vi "Calc phase increase and offset.vi"(6 "Phase offset (deg)":dbl, 7 "# of DDS":i32=4, 8 "error in (no error)":errorcluster, 9 "resolution (32bit)":i32=32, 10 "fclk (MHz)":dbl=800000000.0 format="%#_6p", 11 "f_generated (MHz)":dbl=10.0) -> (0 "error out":errorcluster, 2 "Phase out":fxp<+,64,64>[](array[numeric]), 3 "delta":i64)   [LabVIEW 2025]
doc: "Calculates Phase Increment (\"pinc\") information for DDS core."
panel:
  out "Numeric":dbl
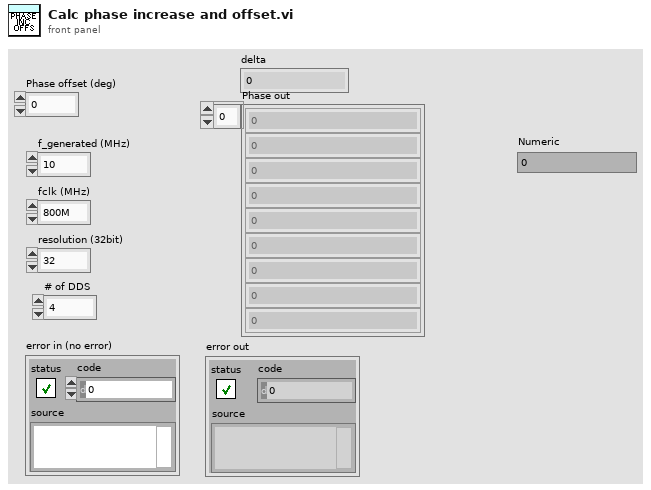
[diagram p1: front panel]
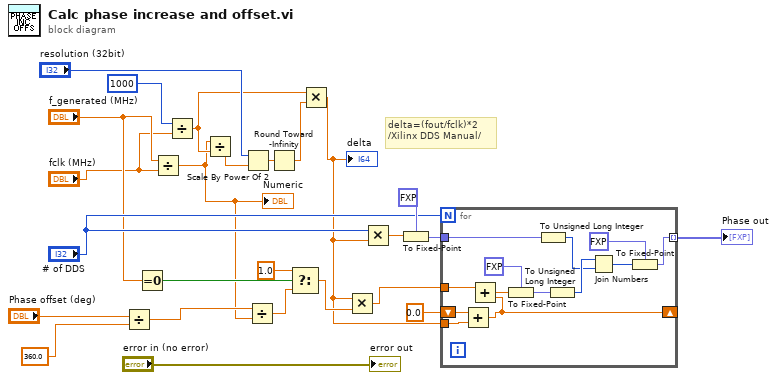
[diagram p0: block diagram]
diagram:
  # "delta=(fout/fclk)*2\n/Xilinx DDS Manual/"
  n1 = Divide(x="Phase offset (deg)", y=360.0) -> (x/y=w17:dbl)
  n2 = Equal To 0?(x="f_generated (MHz)") -> (x = 0?=w11:bool)
  n3 = Divide(x="f_generated (MHz)", y="fclk (MHz)") -> (x/y=w2:dbl)
  "Numeric" <- w2
  n4 = Divide(x=1000, y="fclk (MHz)") -> (x/y=w3:dbl)
  n5 = Divide(x=w2, y=w3) -> (x/y=w7:dbl)
  n6 = Scale By Power Of 2(n="resolution (32bit)", x=w7) -> (x*2^n=w21:dbl)
  n7 = Divide(x=w17, y=w2) -> (x/y=w12:dbl)
  n8 = Round Toward -Infinity(1:w21) -> (0:w4:dbl)
  n9 = Select(t=1.0, s=w11, f=w12) -> (s? t:f=w10:dbl)
  n10 = Multiply(x=w3, y=w4) -> (x*y=w6:dbl)
  "delta" <- w6
  n11 = Multiply(x=w6, y=w10) -> (x*y=w16:dbl)
  n12 = Multiply(x="# of DDS", y=w6) -> (x*y=w14:dbl)
  n13 = To Fixed-Point(fixed-point type=fxp<+,32,32> 0.0 ("pinc_in0"), number=w14) -> (fixed-point=w22:fxp<+,32,32>)
  n14 = for {
    N: "# of DDS" -> [_]
    tunnel: w22 -> [w33]
    tunnel: [w27] -> w19 mode=indexing
    tunnel: w6 -> [w38]
    shift-right: [w35] -> _
    shift-left: 0.0 -> [w36]
    tunnel: w16 -> [w34]
    n15 = Add(x=w36, y=w38) -> (x+y=w35:dbl)
    n16 = Add(x=w34, y=w35) -> (x+y=w26:dbl)
    n17 = To Fixed-Point(fixed-point type=fxp<+,32,32> 0.0 ("pinc_in0"), number=w26) -> (fixed-point=w32:fxp<+,32,32>)
    n18 = To Unsigned Long Integer(number=w33) -> (unsigned 32bit integer=w30:u32)
    n19 = To Unsigned Long Integer(number=w32) -> (unsigned 32bit integer=w31:u32)
    n20 = Join Numbers(hi=w31, lo=w30) -> ((hi.lo)=w29:u64)
    n21 = To Fixed-Point(fixed-point type=fxp<+,64,64> 0.0, number=w29) -> (fixed-point=w27:fxp<+,64,64>)
  }
  "Phase out" <- w19
  "error out" <- "error in (no error)"
